vi "TestTimer.vi"(11 "error in":errorcluster) -> (15 "error out":errorcluster)   [LabVIEW 2016, in "TimerTest.lvlib"]
doc: "Test for Timer"
uses:
  TimerTest.lvlib
  APIs/Stimulus/VI/MakeVIFrontMost.vi
  APIs/Stimulus/ControlValue/ValueSignalLatchBooleanString.vi
  APIs/Assert/AssertControlValue/AlmostEqual.vi
  <vilib>/addons/_JKI Toolkits/Caraya/classes/Assert/Assert Almost Equal_Float.vi
  APIs/Stimulus/ControlValue/SetValueAuto.vi
  APIs/Stimulus/VI/CloseVI.vi
  <vilib>/addons/_JKI Toolkits/Caraya/classes/Test/Test.lvclass
  Drona.lvlib
  APIs/Assert/AssertControlValue/AssertControlValue.lvlib
  APIs/Stimulus/ControlValue/ControlValue.lvlib
  <vilib>/addons/_JKI Toolkits/Caraya/classes/Assert/Assert.lvclass
  APIs/Stimulus/VI/VI.lvlib
panel:
  # "TIMER TEST"
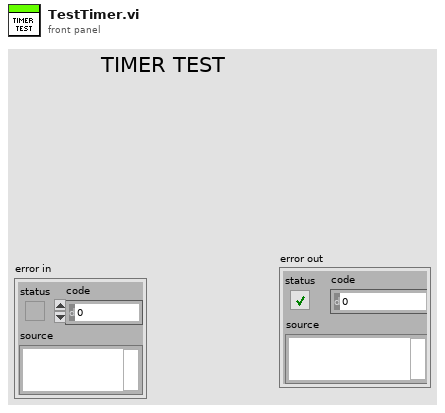
[diagram p1: front panel]
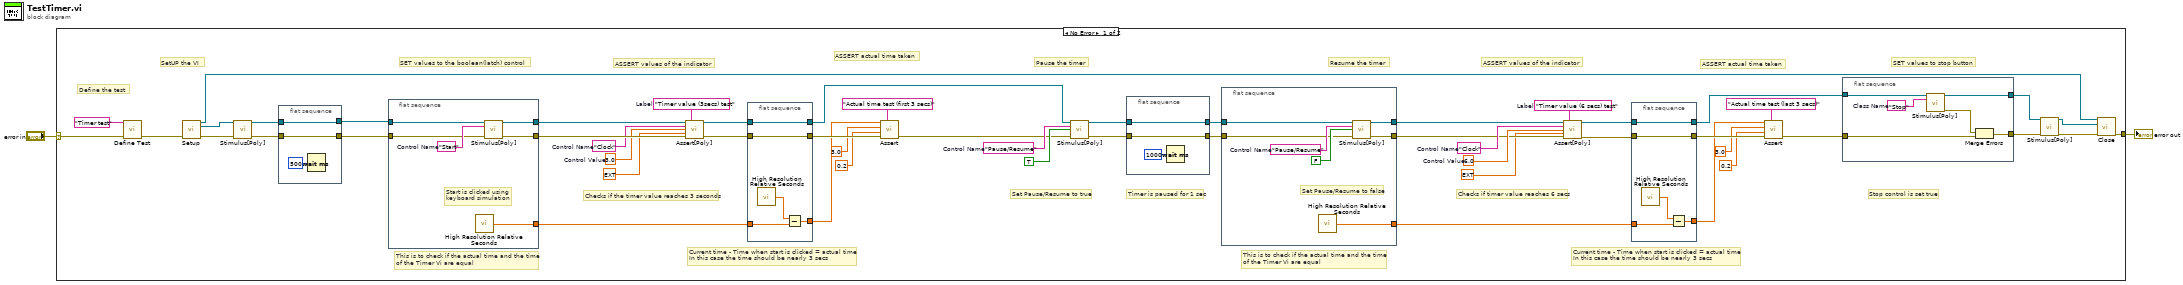
[diagram p0: block diagram]
diagram:
  n1 = case shown="No Error" "error in" {
    selector: "error in" -> [w7 w91]
    tunnel: [w11 w91] -> w2
    frame No Error {
      w46 = "Clock"  # Control Name
      w47 = "Timer value (6 secs) test"  # Label
      w48 = 6.0  # Control Value
      w49 = "Pause/Resume"  # Control Name
      w50 = "Clock"  # Control Name
      w51 = "Timer value (3secs) test"  # Label
      w52 = 3.0  # Control Value
      # "ASSERT actual time taken"
      # "This is to check if the actual time and the time \nof the Timer Vi are equal"
      # "Current time - Time when start is clicked = actual time\nIn this case the time should be nearly 3 secs"
      # "ASSERT actual time taken"
      # "Current time - Time when start is clicked = actual time\nIn this case the time should be nearly 3 secs"
      # "This is to check if the actual time and the time \nof the Timer Vi are equal"
      # "Resume the timer"
      # "Timer is paused for 1 sec"
      # "Checks if timer value reaches 6 secs"
      # "ASSERT values of the indicator"
      # "Stop control is set true"
      # "SET values to stop button"
      # "Set Pause/Resume to true"
      # "Pause the timer"
      # "Checks if the timer value reaches 3 seconds"
      # "ASSERT values of the indicator"
      # "SET values to the boolean(latch) control"
      # "SetUP the VI"
      # "Define the test"
      n2 = call <vilib>:"Define Test.vi"("error in (no error)"=w7, "Label (VI Title)"="Timer test") -> ("error out"=w12:errorcluster)  [unwired: 8 in, 1 out]
      n3 = call "Setup.vi"("error in"=w12) -> ("Application Ref"=w10:refnum<vi>, "VI Reference Out"=w9:refnum<vi>, "error out"=w8:errorcluster)  [unwired: 12 in]
      n4 = call-poly "Stimulus[Poly].vi"("VI Reference In"=w9, "error in"=w8) -> ("VI Reference Out"=w13:refnum<vi>, "error out"=w16:errorcluster)  [unwired: 12 in]
      n5 = flat-sequence {
        tunnel: w16 -> [w57]
        tunnel: [w57] -> w15
        tunnel: [w56] -> w14
        tunnel: w13 -> [w56]
        frame #0 {
          n6 = Wait (ms)(milliseconds to wait=u32 500) -> ()  [unwired: 1 out]
        }
      }
      n7 = flat-sequence {
        tunnel: [w81] -> w54
        tunnel: [w80] -> w53
        tunnel: w15 -> [w78]
        tunnel: w14 -> [w76]
        tunnel: [w77] -> w32
        frame #0 {
          w79 = "Start"  # Control Name
          # "Start is clicked using \nkeyboard simulation"
          n8 = call <vilib>:"High Resolution Relative Seconds.vi"() -> ("relative seconds"=w77:dbl)
          n9 = call-poly "Stimulus[Poly].vi"("VI Reference In"=w76, "Control Path"=w79, "error in"=w78) -> ("VI Reference Out"=w80:refnum<vi>, "error out"=w81:errorcluster)  [unwired: 11 in]
        }
      }
      n10 = call-poly "Assert[Poly].vi"("VI Reference In"=w53, "Test Label"=w51, "Control Path"=w50, "Control Value"=w52, "Tolerance"=ext 0.2, "Error In"=w54) -> ("VI Reference Out"=w34:refnum<vi>, "Error Out"=w36:errorcluster)  [unwired: 7 in, 1 out]
      n11 = flat-sequence {
        tunnel: w36 -> [w75]
        tunnel: [w75] -> w35
        tunnel: w34 -> [w74]
        tunnel: [w74] -> w33
        tunnel: w32 -> [w72]
        tunnel: [w73] -> w30
        frame #0 {
          n12 = call <vilib>:"High Resolution Relative Seconds.vi"() -> ("relative seconds"=w71:dbl)
          n13 = Subtract(x=w71, y=w72) -> (x-y=w73:dbl)
        }
      }
      n14 = call-poly <vilib>:"Assert.vi"("Label"="Actual time test (first 3 secs)", "error in (no error)"=w35, "Tolerance"=0.2, "Y"=3.0, "X"=w30) -> ("error out"=w31:errorcluster)  [unwired: 5 in, 1 out]
      n15 = call-poly "Stimulus[Poly].vi"("VI Reference In"=w33, "Control Path"=w49, "Value (Signaling)"=TRUE, "error in"=w31) -> ("VI Reference Out"=w42:refnum<vi>, "error out"=w43:errorcluster)  [unwired: 10 in]
      n16 = flat-sequence {
        tunnel: w43 -> [w83]
        tunnel: [w83] -> w40
        tunnel: w42 -> [w82]
        tunnel: [w82] -> w41
        frame #0 {
          n17 = Wait (ms)(milliseconds to wait=u32 1000) -> ()  [unwired: 1 out]
        }
      }
      n18 = flat-sequence {
        tunnel: w41 -> [w68]
        tunnel: w40 -> [w67]
        tunnel: [w66] -> w39
        tunnel: [w65] -> w38
        tunnel: [w64] -> w20
        frame #0 {
          w69 = "Pause/Resume"  # Control Name
          # "Set Pause/Resume to false"
          n19 = call <vilib>:"High Resolution Relative Seconds.vi"() -> ("relative seconds"=w64:dbl)
          n20 = call-poly "Stimulus[Poly].vi"("VI Reference In"=w68, "Control Path"=w69, "Value (Signaling)"=FALSE, "error in"=w67) -> ("VI Reference Out"=w65:refnum<vi>, "error out"=w66:errorcluster)  [unwired: 10 in]
        }
      }
      n21 = call-poly "Assert[Poly].vi"("VI Reference In"=w38, "Test Label"=w47, "Control Path"=w46, "Control Value"=w48, "Tolerance"=ext 0.2, "Error In"=w39) -> ("VI Reference Out"=w19:refnum<vi>, "Error Out"=w21:errorcluster)  [unwired: 7 in, 1 out]
      n22 = flat-sequence {
        tunnel: w21 -> [w63]
        tunnel: [w63] -> w26
        tunnel: w19 -> [w62]
        tunnel: [w62] -> w18
        tunnel: w20 -> [w60]
        tunnel: [w61] -> w25
        frame #0 {
          n23 = call <vilib>:"High Resolution Relative Seconds.vi"() -> ("relative seconds"=w59:dbl)
          n24 = Subtract(x=w59, y=w60) -> (x-y=w61:dbl)
        }
      }
      n25 = call-poly <vilib>:"Assert.vi"("Label"="Actual time test (last 3 secs)", "error in (no error)"=w26, "Tolerance"=0.2, "Y"=3.0, "X"=w25) -> ("error out"=w17:errorcluster)  [unwired: 5 in, 1 out]
      n26 = flat-sequence {
        tunnel: [w88] -> w6
        tunnel: [w89] -> w4
        tunnel: w18 -> [w87]
        tunnel: w17 -> [w85]
        frame #0 {
          w90 = "Stop"  # Class Name
          n27 = call-poly "Stimulus[Poly].vi"("VI Reference In"=w87, "Control Path"=w90) -> ("VI Reference Out"=w89:refnum<vi>, "error out"=w86:errorcluster)  [unwired: 12 in]
          n28 = Merge Errors(w86, w85) -> (w88:errorcluster)
        }
      }
      n29 = call-poly "Stimulus[Poly].vi"("VI Reference In"=w4, "error in"=w6) -> ("VI Reference Out"=w3:refnum<vi>, "error out"=w5:errorcluster)  [unwired: 12 in]
      n30 = call "Close.vi"("Application Ref"=w10, "VI Reference"=w3, "error in"=w5) -> ("error out"=w11:errorcluster)  [unwired: 12 in]
    }
    frame Error {
    }
  }
  "error out" <- w2
